vi "Sequence Executor Launcher.vi"() -> ()   [LabVIEW 2026]
doc: "Launcher for the Universal Sequence Executor. Run this VI: it bundles the display refs, launches the executor through Launch Executor, and serves Load / Start / Stop / E-Stop (High priority) / Exit buttons. Exit sends Normal Stop and waits for the Stopped Notification. Use the Exit button to close."
uses:
  src/Executor Messages/Load Sequence Msg/Load Sequence Msg.lvclass/Load Sequence Msg.ctl
  <vilib>/ActorFramework/Message Enqueuer/Message Enqueuer.lvclass/Message Enqueuer.ctl
  <vilib>/ActorFramework/Message Enqueuer/Enqueue.vi
  src/Executor Messages/Load Sequence Msg/Load Sequence Msg.lvclass
  C:/Program Files/National Instruments/LabVIEW 2026/vi.lib/ActorFramework/Message/Message.lvclass
  src/Executor Messages/Start Sequence Msg/Start Sequence Msg.lvclass
  src/Executor Messages/Stop Sequence Msg/Stop Sequence Msg.lvclass
  src/Executor Messages/Emergency Stop Msg/Emergency Stop Msg.lvclass
  <vilib>/ActorFramework/Stop Msg/Stop Msg.lvclass
  <vilib>/ActorFramework/Message Priority Queue/Priority Enqueue.vi
  src/Executor/Sequence Executor.lvclass
panel:
  out "error out":errorcluster
  out "Stopped cleanly":bool
  out "Feedback Chart":dbl
  out "Verdict":string
  out "Channel Values":string[][](array[string])
  out "Step Table":string[][](array[string])
  out "Step Index":i32
  out "Status":string
  in  "Exit":bool
  in  "E-Stop":bool
  in  "Stop":bool
  in  "Start":bool
  in  "Sequence Path":path=path "C:/Users/DynaAdmin/PycharmProjects/Universal-sequence-executor-AF/configs/sequences/vtu_actual_sequence.json"
  in  "Load":bool
  in  "error in":errorcluster
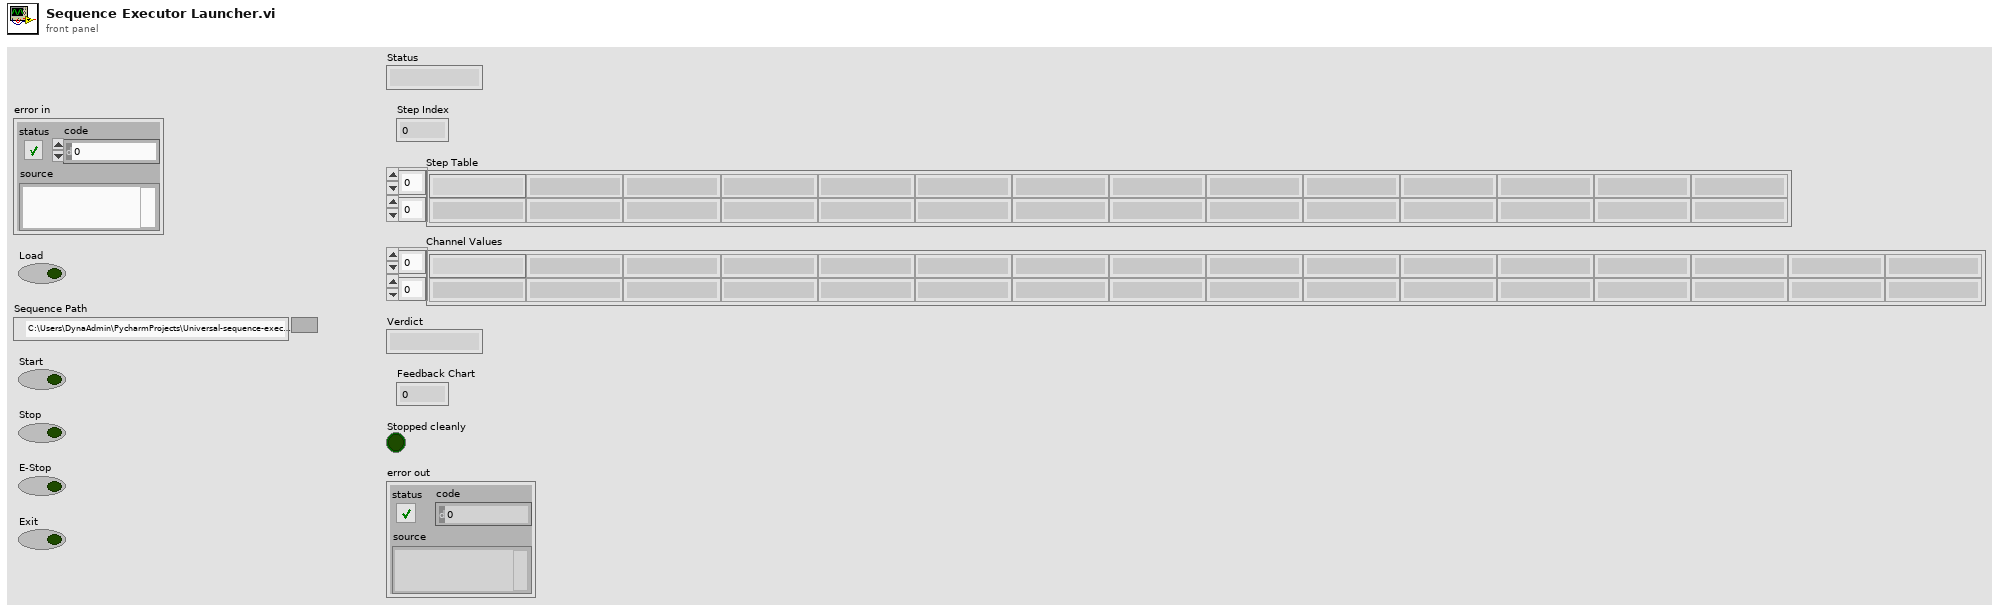
[diagram p1: front panel]
types:
  T1 = cluster{"Status Display":refnum<vi>, "Step Index Display":refnum<vi>, "Step Table Display":refnum<vi>, "Channel Values Display":refnum<vi>, "Verdict Display":refnum<vi>, "Feedback Chart":refnum<vi>}
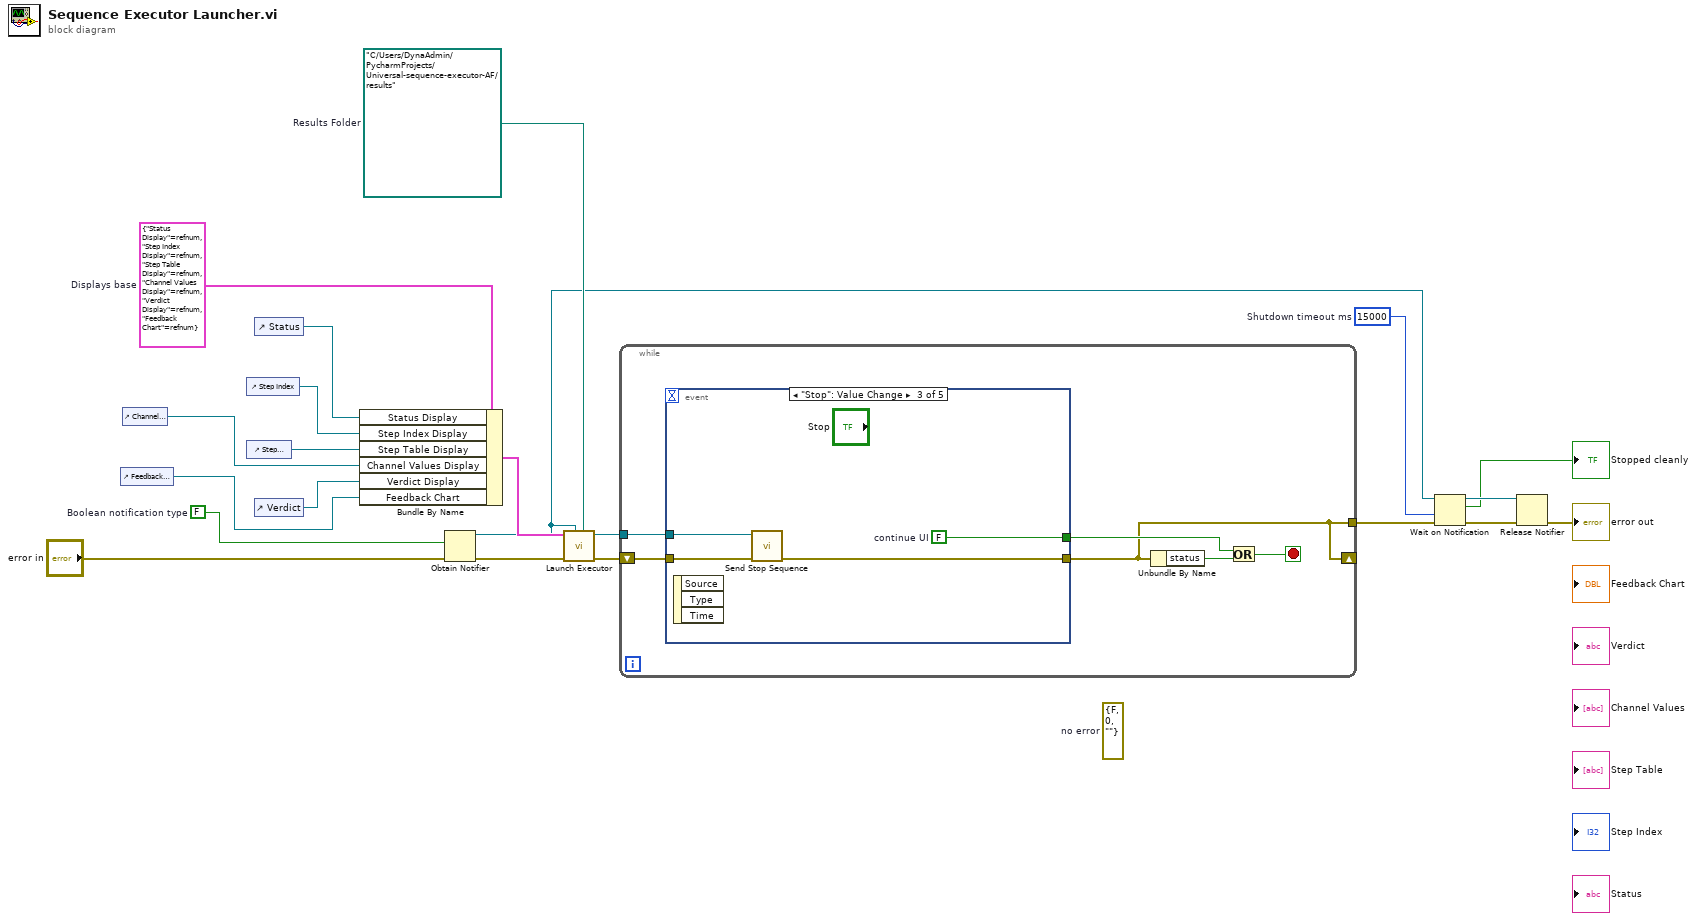
[diagram p0: block diagram]
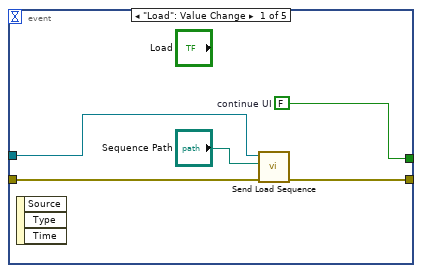
[diagram p2: hidden frame]
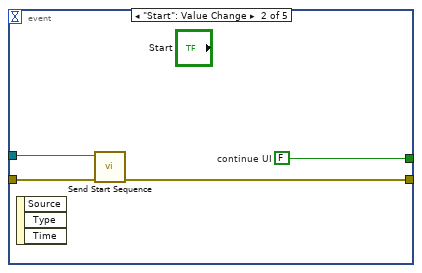
[diagram p3: hidden frame]
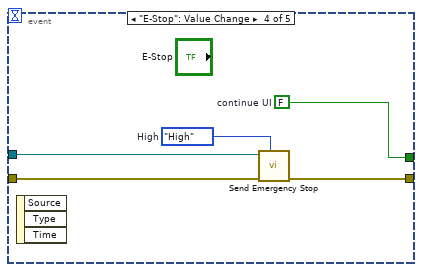
[diagram p4: hidden frame]
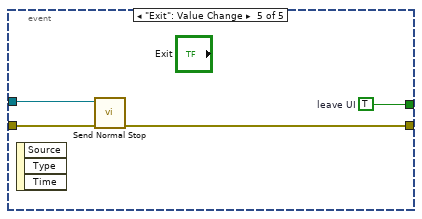
[diagram p5: hidden frame]
diagram:
  w15 = T1 {"Status Display"=refnum, "Step Index Display"=refnum, "Step Table Display"=refnum, "Channel Values Display"=refnum, "Verdict Display"=refnum, "Feedback Chart"=refnum}  # Displays base
  w10 = path "C:/Users/DynaAdmin/PycharmProjects/Universal-sequence-executor-AF/results"  # Results Folder
  w7 = 15000  # Shutdown timeout ms
  (unwired) errorcluster {"status"=FALSE, "code"=0, "source"=""}  # no error
  w14 = FALSE  # Boolean notification type
  n1 = control-ref of="Feedback Chart"() -> (w16:refnum<vi>)
  n2 = control-ref of="Channel Values"() -> (w18:refnum<vi>)
  n3 = control-ref of="Step Index"() -> (w20:refnum<vi>)
  n4 = control-ref of="Step Table"() -> (w19:refnum<vi>)
  n5 = control-ref of="Status"() -> (w21:refnum<vi>)
  n6 = control-ref of="Verdict"() -> (w17:refnum<vi>)
  n7 = Bundle By Name(cluster=w15, "Status Display"=w21, "Step Index Display"=w20, "Step Table Display"=w19, "Channel Values Display"=w18, "Verdict Display"=w17, "Feedback Chart"=w16) -> (w12:T1)
  n8 = Obtain Notifier(notification data type=w14, error in (no error)="error in") -> (notifier out=w8:refnum<notifier>, error out=w11:errorcluster)  [unwired: 2 in, 1 out]
  n9 = call "Launch Executor.vi"("Results Folder"=w10, "Stopped Notification"=w8, "error in"=w11, "Displays"=w12) -> ("error out"=w3:errorcluster, "Enqueuer"=w9:refnum<class "Message Enqueuer.lvclass">)  [unwired: 6 in]
  n10 = while {
    tunnel: w9 -> [w27]
    shift-right: [w22] -> _
    shift-left: w3 -> [w26]
    tunnel: [w22] -> w1
    stop <- w23 stop-if-true
    n11 = event shown="[2] \"Stop\": Value Change" {
      selector: _ -> [_ _ _ _ _]
      dyn-events: _ -> [_ _ _ _ _]
      timeout: _ -> [_ _ _ _ _]
      tunnel: w27 -> [w32 w36 w40 w45 w49]
      tunnel: w26 -> [w30 w35 w39 w44 w48]
      tunnel: [w29 w34 w38 w42 w47] -> w25
      tunnel: [w28 w33 w37 w41 w46] -> w22
      event "Load": Value Change {
        w29 = FALSE  # continue UI
        n12 = event-data() -> ()  [unwired: 1 in, 3 out]
        n13 = call "Send Load Sequence.vi"("error in (no error)"=w30, "path"="Sequence Path", "Message Enqueuer"=w32) -> ("error out"=w28:errorcluster)  [unwired: 7 in, 1 out]
      }
      event "Start": Value Change {
        w34 = FALSE  # continue UI
        n14 = event-data() -> ()  [unwired: 1 in, 3 out]
        n15 = call "Send Start Sequence.vi"("error in (no error)"=w35, "Message Enqueuer"=w36) -> ("error out"=w33:errorcluster)  [unwired: 8 in, 1 out]
      }
      event "Stop": Value Change {
        w38 = FALSE  # continue UI
        n16 = event-data() -> ()  [unwired: 1 in, 3 out]
        n17 = call "Send Stop Sequence.vi"("error in (no error)"=w39, "Message Enqueuer"=w40) -> ("error out"=w37:errorcluster)  [unwired: 8 in, 1 out]
      }
      event "E-Stop": Value Change {
        w42 = FALSE  # continue UI
        w43 = enum16{"Low", "Normal", "High"}."High"  # High
        n18 = event-data() -> ()  [unwired: 1 in, 3 out]
        n19 = call "Send Emergency Stop.vi"("Message Priority (Normal)"=w43, "error in (no error)"=w44, "Message Enqueuer"=w45) -> ("error out"=w41:errorcluster)  [unwired: 7 in, 1 out]
      }
      event "Exit": Value Change {
        w47 = TRUE  # leave UI
        n20 = event-data() -> ()  [unwired: 1 in, 3 out]
        n21 = call <vilib>:"Send Normal Stop.vi"("error in (no error)"=w48, "Message Enqueuer"=w49) -> ("error out"=w46:errorcluster)  [unwired: 9 in]
      }
    }
    n22 = Unbundle By Name(w22) -> ("status"=w24:bool)
    n23 = Or(x=w25, y=w24) -> (x .or. y?=w23:bool)
  }
  n24 = Wait on Notification(notifier=w8, timeout in ms (-1)=w7, error in (no error)=w1) -> (notifier out=w6:refnum<notifier>, notification=→"Stopped cleanly":bool, error out=w2:errorcluster)  [unwired: 1 in, 1 out]
  n25 = Release Notifier(notifier=w6, error in (no error)=w2) -> (error out=→"error out":errorcluster)  [unwired: 1 in, 2 out]
